vi "main_test_lab2_3.vi"() -> ()   [LabVIEW 2025]
uses:
  <vilib>/rvi/DesktopExecutionNode/DesktopExecutionNode.xnode
  <vilib>/rvi/DesktopExecutionNode/Execution/niFpgaDEN_Execute.vi
panel:
  out "Waveform Acc Now":T1(graph)
  out "Waveform Acc Max":T2(graph)
  in  "Shake left":bool
  in  "Shake forward":bool
  out "Mean X":fxp<+/-,64,33>
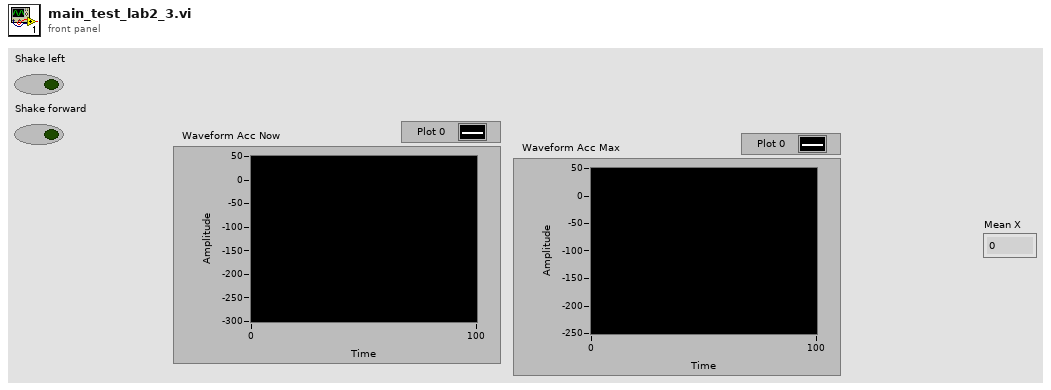
[diagram p1: front panel]
types:
  T1 = cluster{"AccelerationX Now":i16, "AccelerationY Now":i16, "AccelerationZ Now":i16}
  T2 = cluster{"AccelerationX Max":i16, "AccelerationY Max":i16, "AccelerationZ Max":i16}
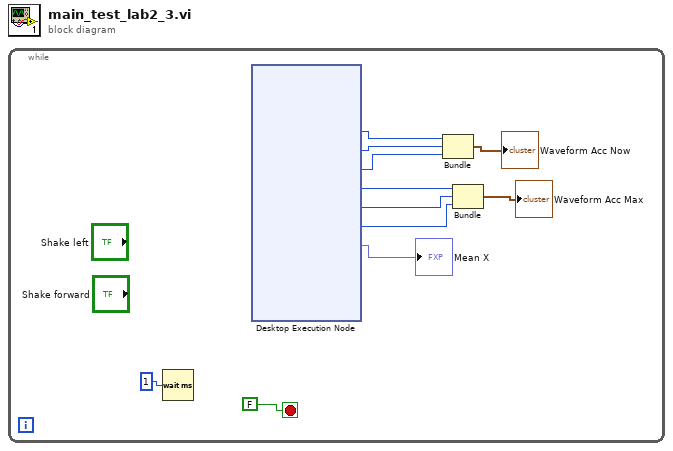
[diagram p0: block diagram]
diagram:
  n1 = while {
    stop <- FALSE stop-if-true
    n2 = Wait (ms)(milliseconds to wait=u32 1) -> ()  [unwired: 1 out]
    n3 = xnode "Desktop Execution Node"() -> ("AccelerationX Now"=w7:i16, "AccelerationY Now"=w6:i16, "AccelerationZ Now"=w5:i16, "AccelerationX Max"=w4:i16, "AccelerationY Max"=w3:i16, "AccelerationZ Max"=w2:i16, "Mean X"=→"Mean X":fxp<+/-,64,33>, "AccelerationZ"=w10:i16, "AccelerationX"=w9:i16, "AccelerationY"=w8:i16)  [unwired: 1 in, 1 out]
    n4 = Bundle("AccelerationX Now"=w7, "AccelerationY Now"=w6, "AccelerationZ Now"=w5) -> (→"Waveform Acc Now":T1)  [unwired: 1 in]
    n5 = Bundle("AccelerationX Max"=w4, "AccelerationY Max"=w3, "AccelerationZ Max"=w2) -> (→"Waveform Acc Max":T2)  [unwired: 1 in]
  }
